vi "global_variant.vi"() -> ()   [LabVIEW 2022 SP3]
panel:
  out "默认路径":path
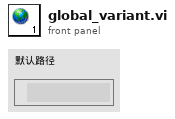
[diagram p1: front panel]
diagram:
